vi "Configure Module.vi"(8 "error in (no error)":errorcluster, 10 "IOV ref in":variant, 11 "9213 in":refnum<class "9213.lvclass">) -> (0 "error out":errorcluster, 2 "IOV ref out":variant, 3 "9213 out":refnum<class "9213.lvclass">)   [LabVIEW 2020, in "Modules.lvlib" / "9213.lvclass"]
uses:
  9213.lvclass
  <resource>/objmgr/cRIO.rc
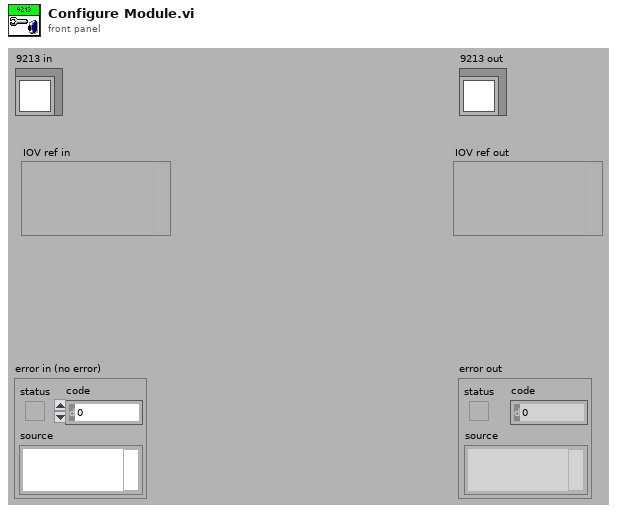
[diagram p1: front panel]
types:
  T1 = typedef "Modules.lvlib/9213.lvclass/Conversion Time.ctl" = u16
  T2 = typedef "Modules.lvlib/9213.lvclass/Measurement Units.ctl" = u8
  T3 = typedef "Modules.lvlib/9213.lvclass/Thermocouple Type.ctl" = u8
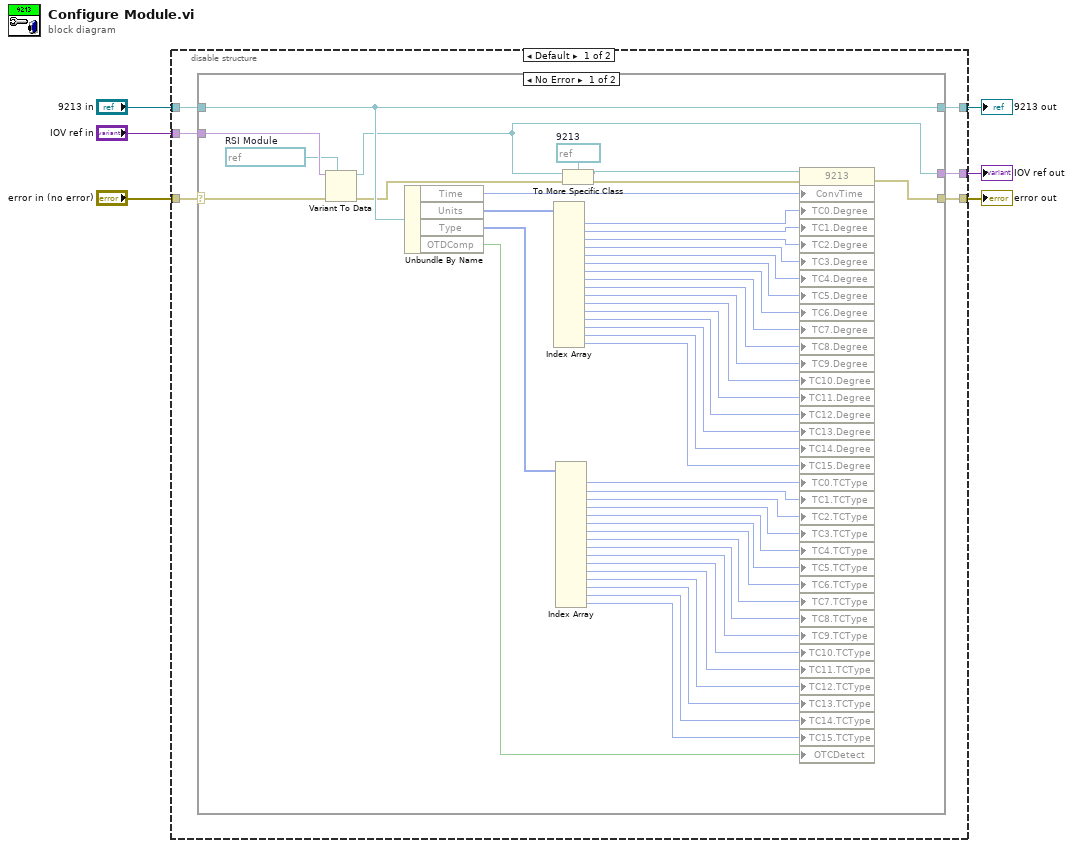
[diagram p0: block diagram]
diagram:
  n1 = disable-structure shown="Default" {
    disable-tunnel: "error in (no error)" -> [w12 w64]
    disable-tunnel: [w11 w64] -> w5
    disable-tunnel: "9213 in" -> [w10 w62]
    disable-tunnel: [w9 w62] -> w3
    disable-tunnel: "IOV ref in" -> [w8 w63]
    disable-tunnel: [w7 w63] -> w1
    frame condition #0 {
      n2 = case shown="No Error" w12 {
        selector: w12 -> [w53 w61]
        tunnel: [w57 w61] -> w11
        tunnel: [w54 w60] -> w9
        tunnel: w10 -> [w54 w60]
        tunnel: w8 -> [w15 w59]
        tunnel: [w14 w59] -> w7
        frame No Error {
          w13 = refnum<k21> refnum  # RSI Module
          w52 = refnum<k21> refnum  # 9213
          n3 = Variant To Data(error in=w53, type=w13, Variant=w15) -> (data=w14:refnum<k21>, error out=w16:errorcluster)
          n4 = Unbundle By Name(w54) -> ("Time"=w58:T1, "Units"=w56:T2[], "Type"=w55:T3[], "OTDComp"=w17:bool)
          n5 = Index Array(array=w56) -> (element #1=w49:T2, element #2=w48:T2, element #3=w47:T2, element #4=w46:T2, element #5=w45:T2, element #6=w44:T2, element #7=w43:T2, element #8=w42:T2, element #9=w41:T2, element #10=w40:T2, element #11=w39:T2, element #12=w38:T2, element #13=w37:T2, element #14=w36:T2, element #15=w35:T2, element #16=w34:T2)  [unwired: 16 in]
          n6 = Index Array(array=w55) -> (element #1=w33:T3, element #2=w32:T3, element #3=w31:T3, element #4=w30:T3, element #5=w29:T3, element #6=w28:T3, element #7=w27:T3, element #8=w26:T3, element #9=w25:T3, element #10=w24:T3, element #11=w23:T3, element #12=w22:T3, element #13=w21:T3, element #14=w20:T3, element #15=w19:T3, element #16=w18:T3)  [unwired: 16 in]
          n7 = To More Specific Class(target class=w52, reference=w14, error in=w16) -> (specific class reference=w51:refnum<k21>, error out=w50:errorcluster)
          n8 = property class="9213"(reference=w51, error in=w50, "ConvTime"=w58, "TC0.Degree"=w49, "TC1.Degree"=w48, "TC2.Degree"=w47, "TC3.Degree"=w46, "TC4.Degree"=w45, "TC5.Degree"=w44, "TC6.Degree"=w43, "TC7.Degree"=w42, "TC8.Degree"=w41, "TC9.Degree"=w40, "TC10.Degree"=w39, "TC11.Degree"=w38, "TC12.Degree"=w37, "TC13.Degree"=w36, "TC14.Degree"=w35, "TC15.Degree"=w34, "TC0.TCType"=w33, "TC1.TCType"=w32, "TC2.TCType"=w31, "TC3.TCType"=w30, "TC4.TCType"=w29, "TC5.TCType"=w28, "TC6.TCType"=w27, "TC7.TCType"=w26, "TC8.TCType"=w25, "TC9.TCType"=w24, "TC10.TCType"=w23, "TC11.TCType"=w22, "TC12.TCType"=w21, "TC13.TCType"=w20, "TC14.TCType"=w19, "TC15.TCType"=w18, "OTCDetect"=w17) -> (error out=w57:errorcluster)  [unwired: 1 out]
        }
        frame Error {
        }
      }
    }
    frame condition #1 (active) {
    }
  }
  "error out" <- w5
  "9213 out" <- w3
  "IOV ref out" <- w1
